vi "Close.vi"(8 "error in (no error)":errorcluster, 11 "ADOResult in":refnum<class "ADOResult.lvclass">) -> (0 "error out":errorcluster)   [LabVIEW 2026, in "ORM_ADONetCore.lvlib" / "ADOResult.lvclass"]
uses:
  ADOResult.lvclass
  ADOResult.lvclass/ADOResult.ctl
  Read Reader.vi
  C:/Program Files/dotnet/shared/Microsoft.NETCore.App/8.0.28/System.Data.Common.dll
  Program Files/dotnet/shared/Microsoft.NETCore.App/8.0.28/System.Data.Common.dll
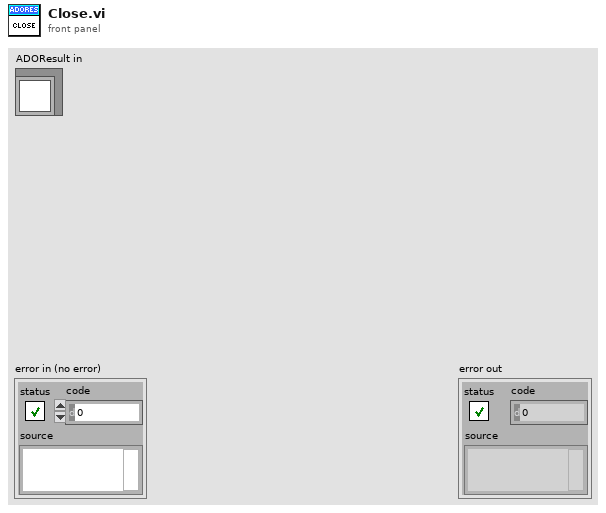
[diagram p1: front panel]
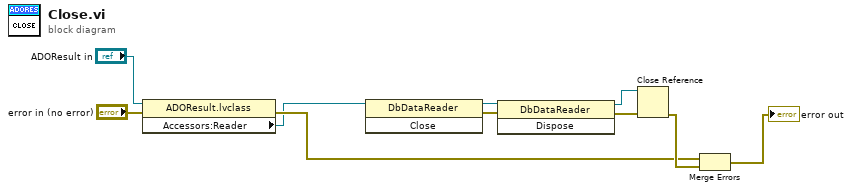
[diagram p0: block diagram]
diagram:
  n1 = property class="ADOResult.lvclass"(reference="ADOResult in", error in="error in (no error)") -> (error out=w3:errorcluster, "Accessors:Reader"=w1:refnum<k39>)  [unwired: 1 out]
  n2 = invoke class="DbDataReader" method="Close"(reference=w1) -> (reference out=w10:refnum<k39>, error out=w9:errorcluster)  [unwired: 2 in, 1 out]
  n3 = invoke class="DbDataReader" method="Dispose"(reference=w10, error in=w9) -> (reference out=w7:refnum<k39>, error out=w8:errorcluster)  [unwired: 1 in, 1 out]
  n4 = Close Reference(reference=w7, error in (no error)=w8) -> (error out=w5:errorcluster)
  n5 = Merge Errors(w3, w5) -> (→"error out":errorcluster)
